vi "LabVIEW.HTTPs_Client.Handle_File.vi"(7 "Command":T1(ring), 8 "Fehler (Eingang, kein Fehler)":errorcluster, 10 "File name":string="Test.csv", 11 "SN":string) -> (0 "Fehler (Ausgang)":errorcluster, 3 "Successful?":bool)   [LabVIEW 2026]
uses:
  <vilib>/Utility/NIReport.llb/NI_report.lvclass
  <vilib>/Utility/NIReport.llb/Report Type.ctl
  <vilib>/Utility/NIReport.llb/NI_ReportGenerationCore.lvlib
  <vilib>/addons/_office/excel.llb/Excel Find and Replace (str).vi
  <vilib>/addons/_office/excel.llb/Excel Get Data (str).vi
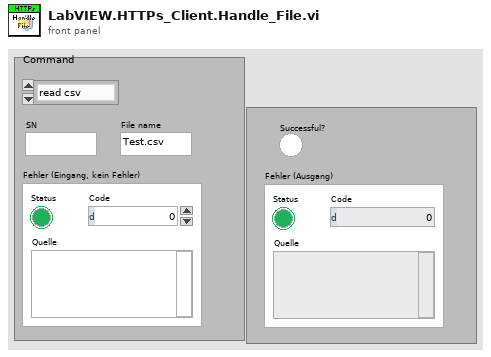
[diagram p1: front panel]
types:
  T1 = enum16{"read csv", "clear csv", "read xlsx", "clear xlsx"}
  T2 = enum16{"maximized", "minimized", "normal", "no change"}
  T3 = typedef "NI_ReportGenerationCore.lvlib/Report Type.ctl" = enum16{"HTML", "Word", "Excel"}
  T4 = enum16{"open", "replace", "create", "open or create", "replace or create", "replace or create with confirmation"}
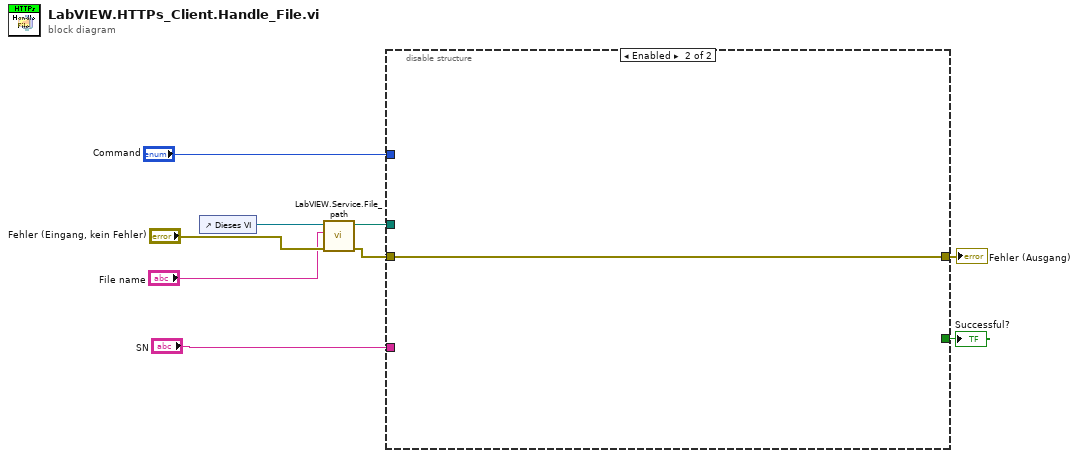
[diagram p0: block diagram]
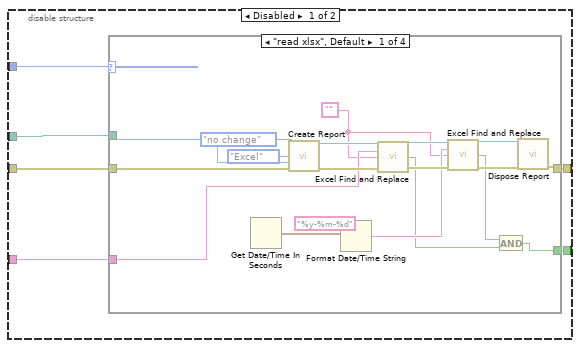
[diagram p2: hidden frame]
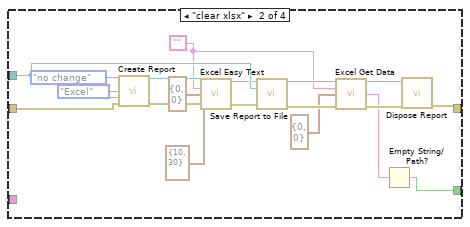
[diagram p3: hidden frame]
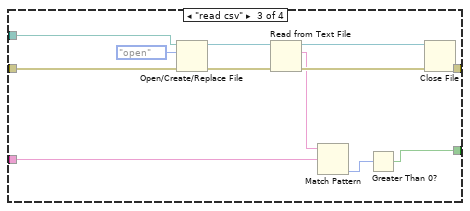
[diagram p4: hidden frame]
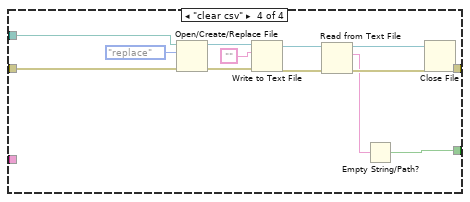
[diagram p5: hidden frame]
diagram:
  n1 = control-ref of="Dieses VI"() -> (w5:refnum<vi>)
  n2 = call "LabVIEW.Service.File_path.vi"("Fehler (Eingang, kein Fehler)"="Fehler (Eingang, kein Fehler)", "File name"="File name", "VI Reference"=w5) -> ("Fehler (Ausgang)"=w2:errorcluster, "Dateipfad-Bedienelement"=w3:path)  [unwired: 7 in]
  n3 = disable-structure shown="Enabled" {
    disable-tunnel: [w15 w79] -> w9
    disable-tunnel: "SN" -> [w14 _]
    disable-tunnel: [w13 _] -> w7
    disable-tunnel: "Command" -> [w12 _]
    disable-tunnel: w3 -> [w11 _]
    disable-tunnel: w2 -> [w10 w79]
    frame Disabled {
      n4 = case shown="\"read xlsx\", Default" w12 {
        tunnel: w11 -> [w33 w49 w65 w78]
        tunnel: w10 -> [w32 w53 w59 w76]
        tunnel: [w31 w51 w58 w75] -> w15
        tunnel: w14 -> [w17 _ w55 _]
        tunnel: [w19 w35 w54 w66] -> w13
        frame "read xlsx", Default {
          w16 = ""
          n5 = Get Date/Time In Seconds() -> (seconds since 1Jan1904=w30:timestamp)
          n6 = call <vilib>:"Create Report.vi"("window state (normal)"=T2."no change", "Report Type"=Report_Type."Excel" ("report type"), "template (empty)"=w33, "error in (no error)"=w32) -> ("report out"=w27:refnum<class "NI_report.lvclass">, "error out"=w28:errorcluster)  [unwired: 10 in]
          n7 = Format Date/Time String(time format string (%c)="%y-%m-%d" ("Zeitformatierungs-String (%c)"), seconds (now)=w30) -> (date/time string=w24:string)  [unwired: 1 in]
          n8 = call-poly <vilib>:"Excel Find and Replace.vi"("report in"=w27, "searched string"=w17, "replacement"=w16, "error in (no error)"=w28) -> ("report out"=w25:refnum<class "NI_report.lvclass">, "found?"=w20:bool, "error out"=w26:errorcluster)  [unwired: 9 in]
          n9 = call-poly <vilib>:"Excel Find and Replace.vi"("report in"=w25, "searched string"=w24, "replacement"=w16, "error in (no error)"=w26) -> ("report out"=w22:refnum<class "NI_report.lvclass">, "found?"=w21:bool, "error out"=w23:errorcluster)  [unwired: 9 in]
          n10 = And(x=w21, y=w20) -> (x .and. y?=w19:bool)
          n11 = call-dynamic "Dispose Report.vi"("report in"=w22, "error in (no error)"=w23) -> ("error out"=w31:errorcluster)  [unwired: 13 in]
        }
        frame "clear xlsx" {
          w38 = ""
          n12 = call <vilib>:"Create Report.vi"("window state (normal)"=T2."no change", "Report Type"=Report_Type."Excel" ("report type"), "template (empty)"=w49, "error in (no error)"=w53) -> ("report out"=w48:refnum<class "NI_report.lvclass">, "error out"=w46:errorcluster)  [unwired: 10 in]
          n13 = call <vilib>:"Excel Easy Text.vi"("report in"=w48, "text"=w38, "start (-1, -1)"=cluster{"row":i32, "column":i32} {"row"=0, "column"=0}, "end (-1, -1)"=cluster{"row":i32, "column":i32} {"row"=10, "column"=30}, "error in (no error)"=w46) -> ("report out"=w47:refnum<class "NI_report.lvclass">, "error out"=w45:errorcluster)  [unwired: 6 in, 3 out]
          n14 = call-dynamic "Save Report to File.vi"("report in"=w47, "report file path"=w49, "error in (no error)"=w45) -> ("report out"=w41:refnum<class "NI_report.lvclass">, "error out"=w42:errorcluster)  [unwired: 11 in]
          n15 = call-poly <vilib>:"Excel Get Data.vi"("report in"=w41, "data type"=w38, "start (0, 0)"=cluster{"start row":i32, "start column":i32} {"start row"=0, "start column"=0}, "error in (no error)"=w42) -> ("report out"=w39:refnum<class "NI_report.lvclass">, "data"=w36:string, "error out"=w40:errorcluster)  [unwired: 9 in]
          n16 = Empty String/Path?(string/path=w36) -> (empty?=w35:bool)
          n17 = call-dynamic "Dispose Report.vi"("report in"=w39, "error in (no error)"=w40) -> ("error out"=w51:errorcluster)  [unwired: 13 in]
        }
        frame "read csv" {
          n18 = Open/Create/Replace File(file path (use dialog)=w65, error in=w59, operation (0:open)=T4."open" ("Operation (0:open)")) -> (refnum out=w63:refnum<file>, error out=w62:errorcluster)  [unwired: 3 in, 1 out]
          n19 = Read from Text File(file (use dialog)=w63, error in=w62) -> (refnum out=w61:refnum<file>, text=w56:string, error out=w60:errorcluster)  [unwired: 2 in, 1 out]
          n20 = Match Pattern(string=w56, regular expression=w55) -> (offset past match=w57:i32)  [unwired: 1 in, 3 out]
          n21 = Greater Than 0?(x=w57) -> (x > 0?=w54:bool)
          n22 = Close File(refnum=w61, error in=w60) -> (error out=w58:errorcluster)  [unwired: 1 out]
        }
        frame "clear csv" {
          n23 = Open/Create/Replace File(file path (use dialog)=w78, error in=w76, operation (0:open)=T4."replace" ("Operation (0:open)")) -> (refnum out=w74:refnum<file>, error out=w73:errorcluster)  [unwired: 3 in, 1 out]
          n24 = Write to Text File(file (use dialog)=w74, text="", error in=w73) -> (refnum out=w71:refnum<file>, error out=w69:errorcluster)  [unwired: 1 in, 1 out]
          n25 = Read from Text File(file (use dialog)=w71, error in=w69) -> (refnum out=w70:refnum<file>, text=w67:string, error out=w68:errorcluster)  [unwired: 2 in, 1 out]
          n26 = Empty String/Path?(string/path=w67) -> (empty?=w66:bool)
          n27 = Close File(refnum=w70, error in=w68) -> (error out=w75:errorcluster)  [unwired: 1 out]
        }
      }
    }
    frame Enabled {
    }
  }
  "Successful?" <- w7
  "Fehler (Ausgang)" <- w9
